vi "UnsyncSource.vi"(5 "Files Generated by Build":path[](array[path]), 6 "Top Level/Always Included VIs":path[](array[path]), 7 "Destination Path":path, 8 "error in (no error)":errorcluster, 9 "Target Name":string, 10 "Build Specification Name":string, 11 "Project Path":path) -> (0 "error out":errorcluster)   [LabVIEW 2023]
panel:
  out "return code":i32
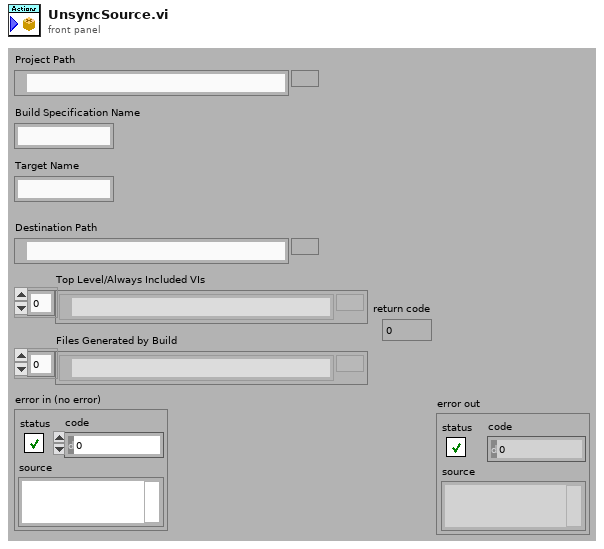
[diagram p1: front panel]
types:
  T1 = enum32{"invalid OS target", "Mac OS", "Windows 3.1", "Windows 95/NT", "Solaris 1", "Solaris 2", "HP-UX", "PowerMAX", "Linux", "Irix", "Rhapsody", "BeOS", "AIX", "OSF1", "VxWorks", "PharLap", "Carbon", "RTX", "Windows x64", "Linux x64"}
  T2 = enum32{"invalid OS target", "Mac OS", "Windows 3.1", "Windows 95/NT", "Solaris 1", "Solaris 2", "HP-UX", "PowerMAX", "Linux", "Irix", "Rhapsody", "BeOS", "AIX", "OSF1", "VxWorks", "PharLap", "Carbon", "RTX", "Windows x64", "Linux x64", "Mac OS X x64", "Windows ARM64", "Linux ARM64", "Mac OS X ARM64"}
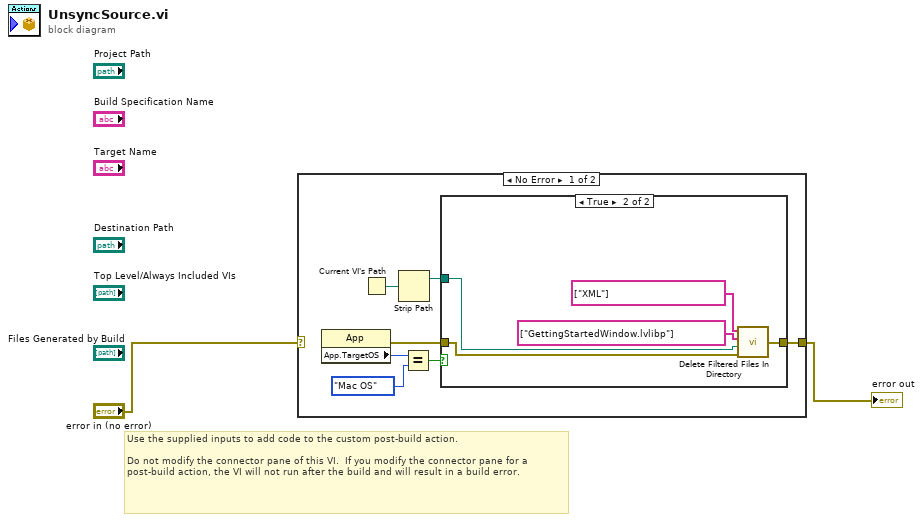
[diagram p0: block diagram]
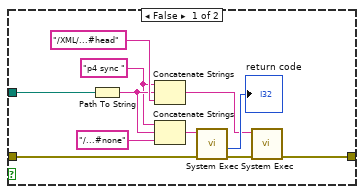
[diagram p2: hidden frame]
diagram:
  # "Use the supplied inputs to add code to the custom post-build action.\n\nDo not modify the connector pane of this VI.  If you modify the connector pane for a post-build action, the VI will not run after the build and will result in a build error."
  n1 = case shown="No Error" "error in (no error)" {
    selector: "error in (no error)" -> [_ w26]
    tunnel: [w8 w26] -> w1
    frame No Error {
      n2 = property class="App"() -> (error out=w7:errorcluster, "App.TargetOS"=w5:T2)  [unwired: 2 in, 1 out]
      n3 = Current VI's Path() -> (path=w9:path)
      n4 = Strip Path(path=w9) -> (stripped path=w3:path)  [unwired: 1 out]
      n5 = Equal?(x=w5, y=T1."Mac OS" ("Application:Target:Operating System")) -> (x = y?=w4:bool)
      n6 = case shown="True" w4 {
        tunnel: [w11 w24] -> w8
        tunnel: w3 -> [w12 w22]
        tunnel: w7 -> [w10 w21]
        frame False {
          w13 = "p4 sync " ("string")
          n7 = Path To String(path=w12) -> (string=w15:string)
          n8 = Concatenate Strings(w13, w15, "/XML/...#head" ("string")) -> (w16:string)
          n9 = Concatenate Strings(w13, w15, "/...#none" ("string")) -> (w20:string)
          n10 = call <vilib>:"System Exec.vi"("error in (no error)"=w10, "command line"=w20) -> ("error out"=w14:errorcluster, "return code"=→"return code":i32)  [unwired: 6 in, 2 out]
          n11 = call <vilib>:"System Exec.vi"("error in (no error)"=w14, "command line"=w16) -> ("error out"=w11:errorcluster)  [unwired: 6 in, 3 out]
        }
        frame True {
          n12 = call <resource>:"Delete Filtered Files In Directory.vi"("Error in"=w21, "Path"=w22, "Files to Exclude"=string[] ["GettingStartedWindow.lvlibp"], "Folders to Exclude"=string[] ["XML"]) -> ("Error out"=w24:errorcluster)
        }
      }
    }
    frame Error {
    }
  }
  "error out" <- w1
